vi "VIH Constant - Product Info Store.vi"() -> (0 "Product Info":T1={"Product Name"="VI Helpeks", "Short Name"="VI Helpeks", "Product Version"="3.1.0", "Release Timestamp"="22-10-2026 08:16:38", "Developer"="Konstantin Shifershteyn", "Copyright"="Copyright (c) 2012-2026, Konstantin Shifershteyn"})   [LabVIEW 2014]
doc: "Product Info Container. The current product info:\nProduct name: VI Helpeks\nShort name: VI Helpeks\nVersion: 3.1.0\nRelease TS: 22-10-2026 08:16:38\nCompany: Konstantin Shifershteyn\nDeveloper(s): Copyright (c) 2012-2026, Konstantin Shifershteyn\nLabVIEW ver: 14.0.1f11"
panel:
  # "VI Helpeks\nCopyright (c) 2012-2026 Konstantin Shifershteyn"
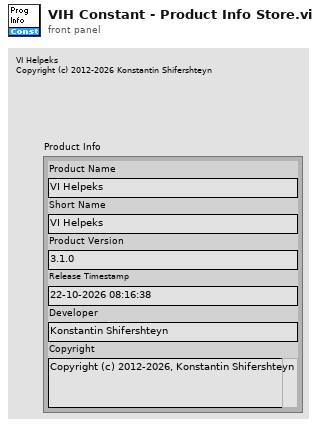
[diagram p1: front panel]
types:
  T1 = cluster{"Product Name":string, "Short Name":string, "Product Version":string, "Release Timestamp":string, "Developer":string, "Copyright":string}
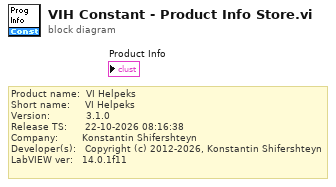
[diagram p0: block diagram]
diagram:
  # "Product name:  VI Helpeks\nShort name:     VI Helpeks\nVersion:            3.1.0\nRelease TS:      22-10-2026 08:16:38\nCompany:        Konstantin Shifershteyn\nDeveloper(s):   Copyright (c) 2012-2026, Konstantin Shifershteyn\nLabVIEW ver:   14.0.1f11"
